vi "CobotCommunicationProtocal.vi"(0 "address":string, 1 "협동로봇 통신 시작":bool, 2 "협동로봇 통신 리셋":bool, 3 "협동로봇 통신 정지":bool, 4 "정지":bool, 5 "Error In":errorcluster caption="에러 입력") -> (6 "상태":T1, 9 "Robot State":u16[](array[numeric]), 11 "Joint Torque":dbl[](array[numeric]), 13 "External Force":dbl[](array[numeric]), 14 "Joint Poistion":dbl[](array[numeric]), 15 "Task Position":dbl[](array[numeric]), 16 "Joint Current":dbl[](array[numeric]), 17 "Joint Temperature":dbl[](array[numeric]), 19 "Error Out":errorcluster caption="에러 출력")   [LabVIEW 2019]
uses:
  ModBusValue.ctl
  <vilib>/NI/Modbus Library/API/Wrapper/Create TCP Master.vi
  <vilib>/NI/Modbus Library/API/Master/Modbus Master.lvclass
  <vilib>/NI/Modbus Library/API/Wrapper/API Main.lvlib
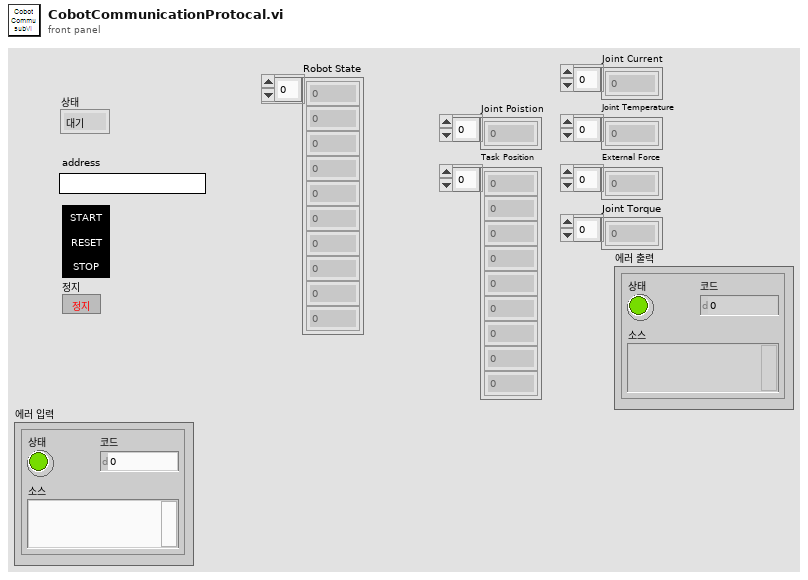
[diagram p1: front panel]
types:
  T1 = typedef "ModBusValue.ctl" = enum16{"대기", "초기화", "읽기", "정지"}
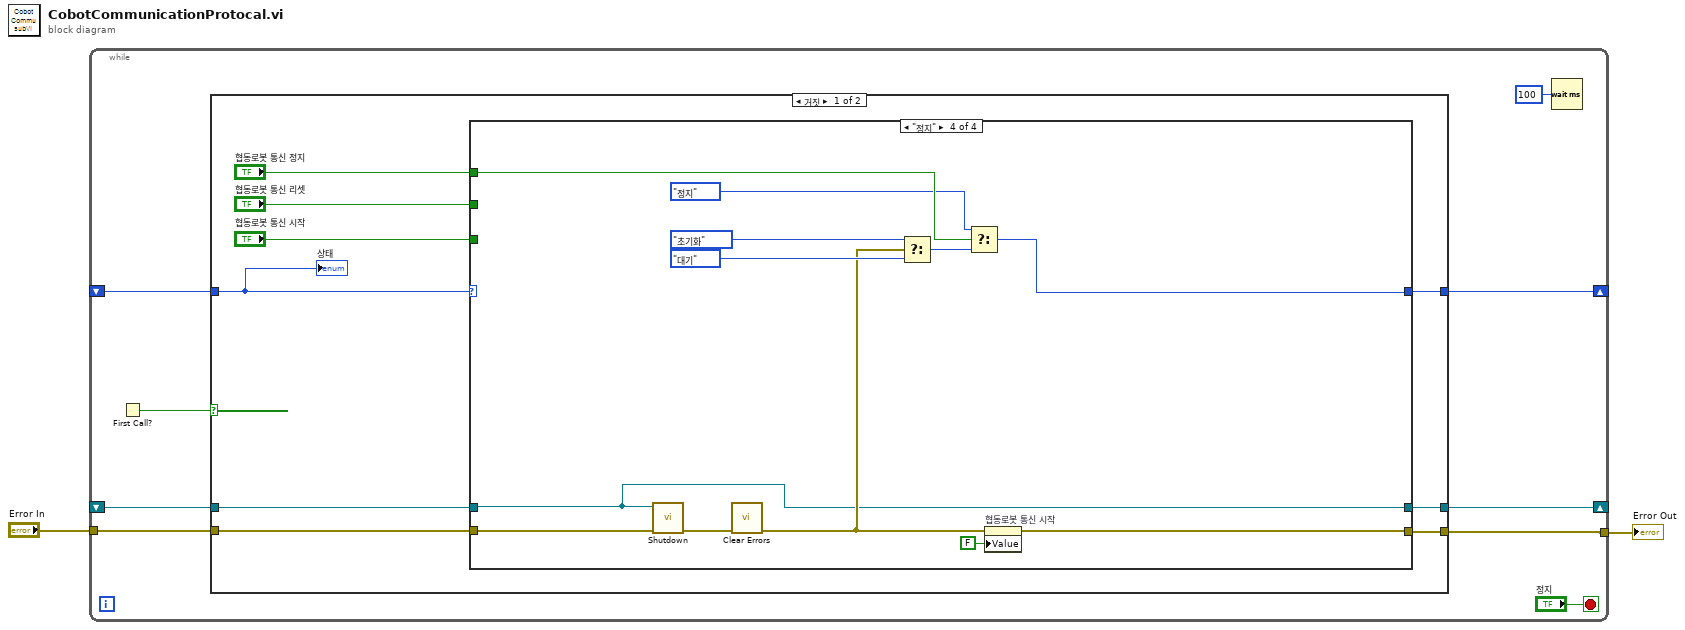
[diagram p0: block diagram]
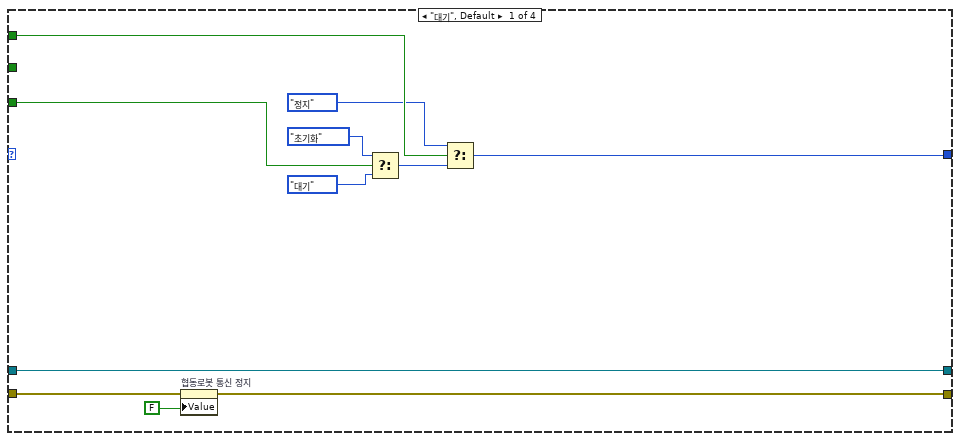
[diagram p2: hidden frame]
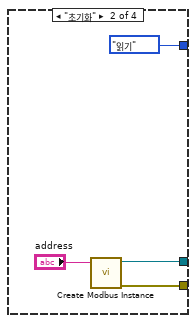
[diagram p3: hidden frame]
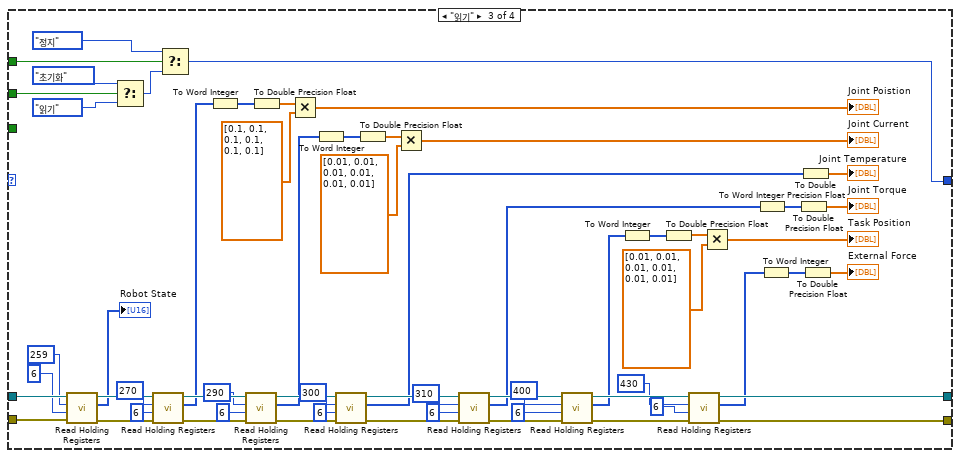
[diagram p4: hidden frame]
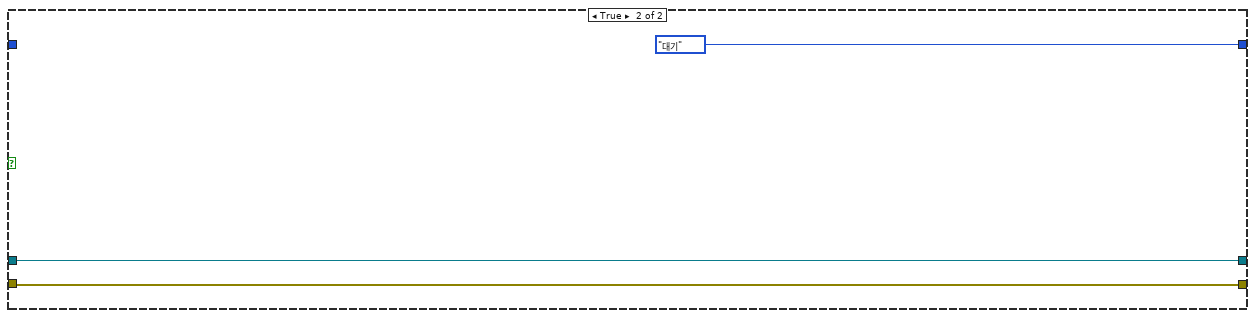
[diagram p5: hidden frame]
diagram:
  n1 = while {
    tunnel: [w8] -> w1
    tunnel: "Error In" -> [w5]
    shift-right: [w10] -> _
    shift-left: _ -> [w9]
    shift-right: [w7] -> _
    shift-left: _ -> [w6]
    stop <- "정지" stop-if-true
    n2 = First Call?() -> (First Call?: T/F=w11:bool)
    n3 = case shown="거짓" w11 {
      tunnel: [w16 ModBusValue."대기" ("열거형")] -> w10
      tunnel: w9 -> [w12 _]
      tunnel: [w17 w109] -> w8
      tunnel: [w15 w110] -> w7
      tunnel: w6 -> [w14 w110]
      tunnel: w5 -> [w13 w109]
      frame False {
        n4 = case shown="\"정지\"" w12 {
          tunnel: "협동로봇 통신 시작" -> [w25 _ _ _]
          tunnel: "협동로봇 통신 리셋" -> [_ _ w40 _]
          tunnel: "협동로봇 통신 정지" -> [w31 _ w41 w107]
          tunnel: [w22 w35 w89 w97] -> w15
          tunnel: [w23 w34 w81 w99] -> w17
          tunnel: [w28 ModBusValue."읽기" ("열거형") w36 w101] -> w16
          tunnel: w14 -> [w22 _ w96 w97]
          tunnel: w13 -> [w24 _ w88 w106]
          frame "대기", Default {
            n5 = property on="협동로봇 통신 정지" class="Bool (엄격한)"(error in=w24, "Value"=FALSE) -> (error out=w23:errorcluster)  [unwired: 1 in, 1 out]
            n6 = Select(t=ModBusValue."초기화" ("열거형"), s=w25, f=ModBusValue."대기" ("열거형")) -> (s? t:f=w29:T1)
            n7 = Select(t=ModBusValue."정지" ("열거형"), s=w31, f=w29) -> (s? t:f=w28:T1)
          }
          frame "초기화" {
            n8 = call-poly <vilib>:"Create Modbus Instance.vi"("address"="address") -> ("error out"=w34:errorcluster, "TCP master instance"=w35:refnum<class "Modbus Master.lvclass">)  [unwired: 9 in]
          }
          frame "읽기" {
            n9 = call-dynamic "Read Holding Registers.vi"("error in"=w88, "number of inputs"=u16 6, "starting address"=u16 259, "Modbus master in"=w96) -> ("error out"=w87:errorcluster, "register values"=→"Robot State":u16[], "Modbus master out"=w95:refnum<class "Modbus Master.lvclass">)  [unwired: 5 in]
            n10 = Select(t=ModBusValue."초기화" ("열거형"), s=w40, f=ModBusValue."읽기" ("열거형")) -> (s? t:f=w42:T1)
            n11 = call-dynamic "Read Holding Registers.vi"("error in"=w87, "number of inputs"=u16 6, "starting address"=u16 270, "Modbus master in"=w95) -> ("error out"=w86:errorcluster, "register values"=w75:u16[], "Modbus master out"=w94:refnum<class "Modbus Master.lvclass">)  [unwired: 5 in]
            n12 = Select(t=ModBusValue."정지" ("열거형"), s=w41, f=w42) -> (s? t:f=w36:T1)
            n13 = To Word Integer(number=w75) -> (16bit integer=w74:i16[])
            n14 = call-dynamic "Read Holding Registers.vi"("error in"=w86, "number of inputs"=u16 6, "starting address"=u16 290, "Modbus master in"=w94) -> ("error out"=w85:errorcluster, "register values"=w67:u16[], "Modbus master out"=w93:refnum<class "Modbus Master.lvclass">)  [unwired: 5 in]
            n15 = To Double Precision Float(number=w74) -> (double precision float=w73:dbl[])
            n16 = Multiply(x=w73, y=dbl[] [0.1, 0.1, 0.1, 0.1, 0.1, 0.1]) -> (x*y=→"Joint Poistion":dbl[])
            n17 = To Word Integer(number=w67) -> (16bit integer=w68:i16[])
            n18 = call-dynamic "Read Holding Registers.vi"("error in"=w85, "number of inputs"=u16 6, "starting address"=u16 300, "Modbus master in"=w93) -> ("error out"=w84:errorcluster, "register values"=w61:u16[], "Modbus master out"=w92:refnum<class "Modbus Master.lvclass">)  [unwired: 5 in]
            n19 = To Double Precision Float(number=w68) -> (double precision float=w69:dbl[])
            n20 = Multiply(x=w69, y=dbl[] [0.01, 0.01, 0.01, 0.01, 0.01, 0.01]) -> (x*y=→"Joint Current":dbl[])
            n21 = call-dynamic "Read Holding Registers.vi"("error in"=w84, "number of inputs"=u16 6, "starting address"=u16 310, "Modbus master in"=w92) -> ("error out"=w83:errorcluster, "register values"=w57:u16[], "Modbus master out"=w91:refnum<class "Modbus Master.lvclass">)  [unwired: 5 in]
            n22 = call-dynamic "Read Holding Registers.vi"("error in"=w83, "number of inputs"=u16 6, "starting address"=u16 400, "Modbus master in"=w91) -> ("error out"=w82:errorcluster, "register values"=w48:u16[], "Modbus master out"=w90:refnum<class "Modbus Master.lvclass">)  [unwired: 5 in]
            n23 = To Word Integer(number=w48) -> (16bit integer=w50:i16[])
            n24 = To Double Precision Float(number=w50) -> (double precision float=w51:dbl[])
            n25 = call-dynamic "Read Holding Registers.vi"("error in"=w82, "number of inputs"=u16 6, "starting address"=u16 430, "Modbus master in"=w90) -> ("error out"=w81:errorcluster, "register values"=w46:u16[], "Modbus master out"=w89:refnum<class "Modbus Master.lvclass">)  [unwired: 5 in]
            n26 = Multiply(x=w51, y=dbl[] [0.01, 0.01, 0.01, 0.01, 0.01, 0.01]) -> (x*y=→"Task Position":dbl[])
            n27 = To Word Integer(number=w57) -> (16bit integer=w56:i16[])
            n28 = To Word Integer(number=w46) -> (16bit integer=w47:i16[])
            n29 = To Double Precision Float(number=w56) -> (double precision float=→"Joint Torque":dbl[])
            n30 = To Double Precision Float(number=w61) -> (double precision float=→"Joint Temperature":dbl[])
            n31 = To Double Precision Float(number=w47) -> (double precision float=→"External Force":dbl[])
          }
          frame "정지" {
            n32 = call-dynamic "Shutdown.vi"("error in"=w106, "Modbus master in"=w97) -> ("error out"=w105:errorcluster)  [unwired: 9 in]
            n33 = call <vilib>:"Clear Errors.vi"("error in (no error)"=w105) -> ("error out"=w100:errorcluster)  [unwired: 5 in, 1 out]
            n34 = Select(t=ModBusValue."초기화" ("열거형"), s=w100, f=ModBusValue."대기" ("열거형")) -> (s? t:f=w108:T1)
            n35 = Select(t=ModBusValue."정지" ("열거형"), s=w107, f=w108) -> (s? t:f=w101:T1)
            n36 = property on="협동로봇 통신 시작" class="Bool (엄격한)"(error in=w100, "Value"=FALSE ("협동로봇 통신 시작")) -> (error out=w99:errorcluster)  [unwired: 1 in, 1 out]
          }
        }
        "상태" <- w12
      }
      frame True {
      }
    }
    n37 = Wait (ms)(milliseconds to wait=u32 100 ("대기 시간 (ms)")) -> ()  [unwired: 1 out]
  }
  "Error Out" <- w1
